vi "Enemies_Blit.vi"(0 "Picture":u8[][](array[numeric]), 1 "View":T1={"Hide"=FALSE, "CX"=0, "CY"=0, "ClaudeIdx"=-1, "ClaudeX"=0, "ClaudeY"=0}, 5 "Sprites":cluster{"Pix":u8[][], "Mask":u8[][]}[](array[cluster]), 7 "Enemies":T2(array[cluster]), 9 "Tick":u32, 11 "error in":errorcluster) -> (4 "Picture out":u8[][](array[numeric]), 15 "error out":errorcluster)   [LabVIEW 2020, in "GH_Render.lvlib"]
doc: "Draws all enemies: spider (legs move every 8 ticks), snake (head sways), skull (turns while rolling). Hide = dark room: only enemies within the light (distance^2 <= 28 tiles)."
uses:
  GH_Render.lvlib
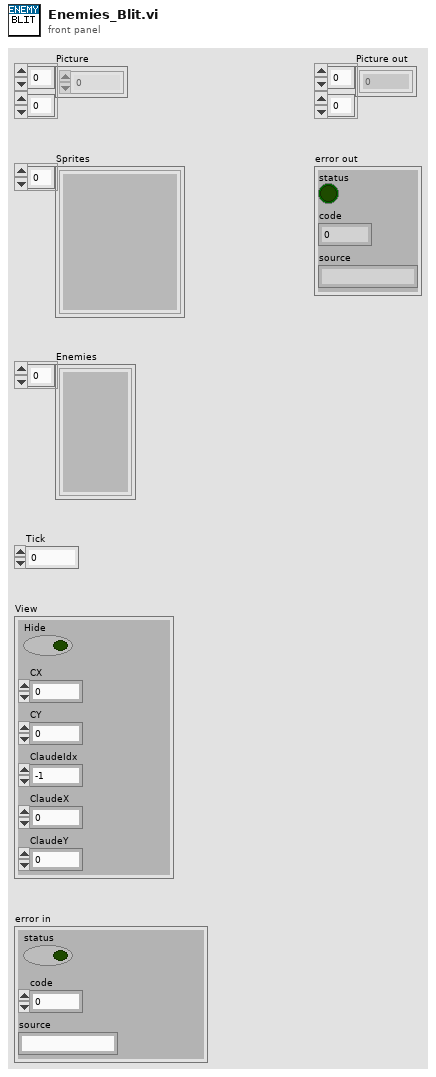
[diagram p1: front panel]
types:
  T1 = cluster{"Hide":bool, "CX":i32, "CY":i32, "ClaudeIdx":i32, "ClaudeX":i32, "ClaudeY":i32}
  T2 = cluster{"Kind":i32, "X10":i32, "Y10":i32, "Dir":i32, "Mode":i32}[]
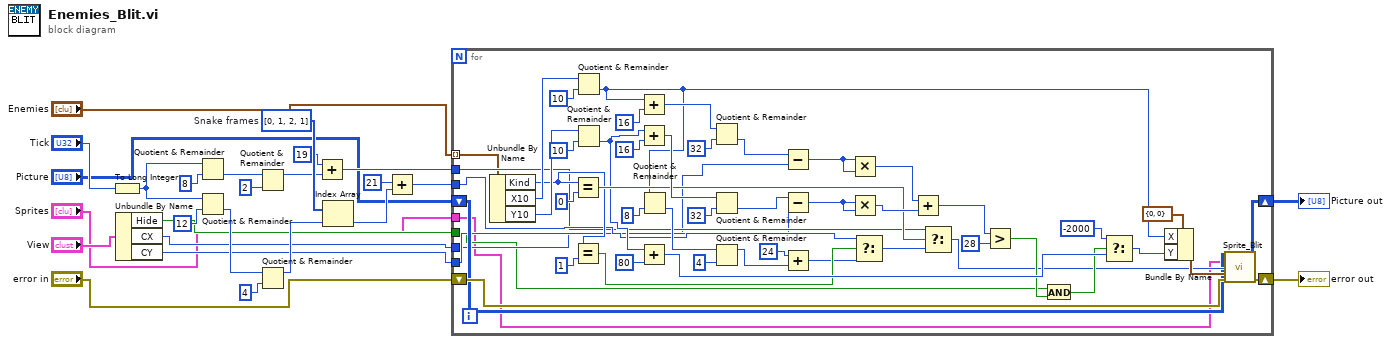
[diagram p0: block diagram]
diagram:
  w18 = i32[] [0, 1, 2, 1]  # Snake frames
  n1 = To Long Integer(number="Tick") -> (32bit integer=w10:i32)
  n2 = Unbundle By Name("View") -> ("Hide"=w7:bool, "CX"=w8:i32, "CY"=w9:i32)
  n3 = Quotient & Remainder(x=w10, y=8) -> (floor(x/y)=w13:i32)  [unwired: 1 out]
  n4 = Quotient & Remainder(x=w10, y=12) -> (floor(x/y)=w20:i32)  [unwired: 1 out]
  n5 = Quotient & Remainder(x=w13, y=2) -> (x-y*floor(x/y)=w15:i32)  [unwired: 1 out]
  n6 = Quotient & Remainder(x=w20, y=4) -> (x-y*floor(x/y)=w22:i32)  [unwired: 1 out]
  n7 = Add(x=19, y=w15) -> (x+y=w16:i32)
  n8 = Index Array(array=w18, index=w22) -> (element=w23:i32)
  n9 = Add(x=21, y=w23) -> (x+y=w24:i32)
  n10 = for {
    tunnel: "Enemies" -> [w27] mode=indexing
    tunnel: "Sprites" -> [w28]
    shift-right: [w35] -> w25
    shift-left: "Picture" -> [w34]
    shift-right: [w37] -> w26
    shift-left: "error in" -> [w36]
    tunnel: w7 -> [w29]
    tunnel: w8 -> [w30]
    tunnel: w9 -> [w31]
    tunnel: w16 -> [w32]
    tunnel: w24 -> [w33]
    n11 = Unbundle By Name(w27) -> ("Kind"=w38:i32, "X10"=w39:i32, "Y10"=w40:i32)
    n12 = Equal?(x=w38, y=0) -> (x = y?=w52:bool)
    n13 = Equal?(x=w38, y=1) -> (x = y?=w54:bool)
    n14 = Quotient & Remainder(x=w39, y=10) -> (floor(x/y)=w42:i32)  [unwired: 1 out]
    n15 = Quotient & Remainder(x=w40, y=10) -> (floor(x/y)=w44:i32)  [unwired: 1 out]
    n16 = Add(x=w42, y=16) -> (x+y=w58:i32)
    n17 = Add(x=w44, y=16) -> (x+y=w63:i32)
    n18 = Add(x=w44, y=80) -> (x+y=w76:i32)
    n19 = Quotient & Remainder(x=w42, y=8) -> (floor(x/y)=w47:i32)  [unwired: 1 out]
    n20 = Quotient & Remainder(x=w58, y=32) -> (floor(x/y)=w60:i32)  [unwired: 1 out]
    n21 = Quotient & Remainder(x=w63, y=32) -> (floor(x/y)=w65:i32)  [unwired: 1 out]
    n22 = Quotient & Remainder(x=w47, y=4) -> (x-y*floor(x/y)=w49:i32)  [unwired: 1 out]
    n23 = Subtract(x=w60, y=w30) -> (x-y=w61:i32)
    n24 = Subtract(x=w65, y=w31) -> (x-y=w66:i32)
    n25 = Add(x=24, y=w49) -> (x+y=w50:i32)
    n26 = Multiply(x=w61, y=w61) -> (x*y=w67:i32)
    n27 = Multiply(x=w66, y=w66) -> (x*y=w68:i32)
    n28 = Select(t=w33, s=w54, f=w50) -> (s? t:f=w55:i32)
    n29 = Add(x=w67, y=w68) -> (x+y=w69:i32)
    n30 = Select(t=w32, s=w52, f=w55) -> (s? t:f=w56:i32)
    n31 = Greater?(x=w69, y=28) -> (0:w71:bool)
    n32 = And(x=w29, y=w71) -> (x .and. y?=w72:bool)
    n33 = Select(t=-2000, s=w72, f=w76) -> (s? t:f=w77:i32)
    n34 = Bundle By Name(cluster=cluster{"X":i32, "Y":i32} {"X"=0, "Y"=0}, "X"=w42, "Y"=w77) -> (w78:cluster{"X":i32, "Y":i32})
    n35 = call "Sprite_Blit.vi"("Picture"=w34, "Sprites"=w28, "Index"=w56, "Position"=w78, "error in"=w36) -> ("Picture out"=w35:u8[][], "error out"=w37:errorcluster)  [unwired: 9 in]
  }
  "Picture out" <- w25
  "error out" <- w26
